vi "RestartSafety.vi"(0 "Universal Robot.lvclass in":refnum<class "Universal Robot.lvclass">, 5 "error in (no error)":errorcluster) -> (14 "Universal Robot.lvclass out":refnum<class "Universal Robot.lvclass">, 19 "error out":errorcluster)   [LabVIEW 2019, in "Universal Robot.lvclass"]
uses:
  Universal Robot.lvclass
  Universal Robot.lvclass/Universal Robot.ctl
  SafetyStatus.ctl
  Client Interfaces/Dashboard Server/Dashboard Server.lvclass
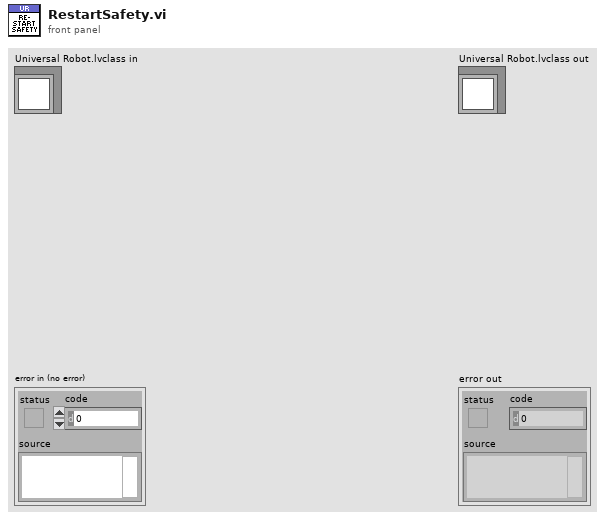
[diagram p1: front panel]
types:
  T1 = typedef "Universal Robot.lvclass/SafetyStatus.ctl" = enum16{"INVALID", "NORMAL", "REDUCED", "PROTECTIVE_STOP", "RECOVERY", "SAFEGUARD_STOP", "SYSTEM_EMERGENCY_STOP", "ROBOT_EMERGENCY_STOP", "VIOLATION", "FAULT", "AUTOMATIC_MODE_SAFEGAURD_STOP", "SYSTEM_THREE_POSITION_ENABLING_STOP"}
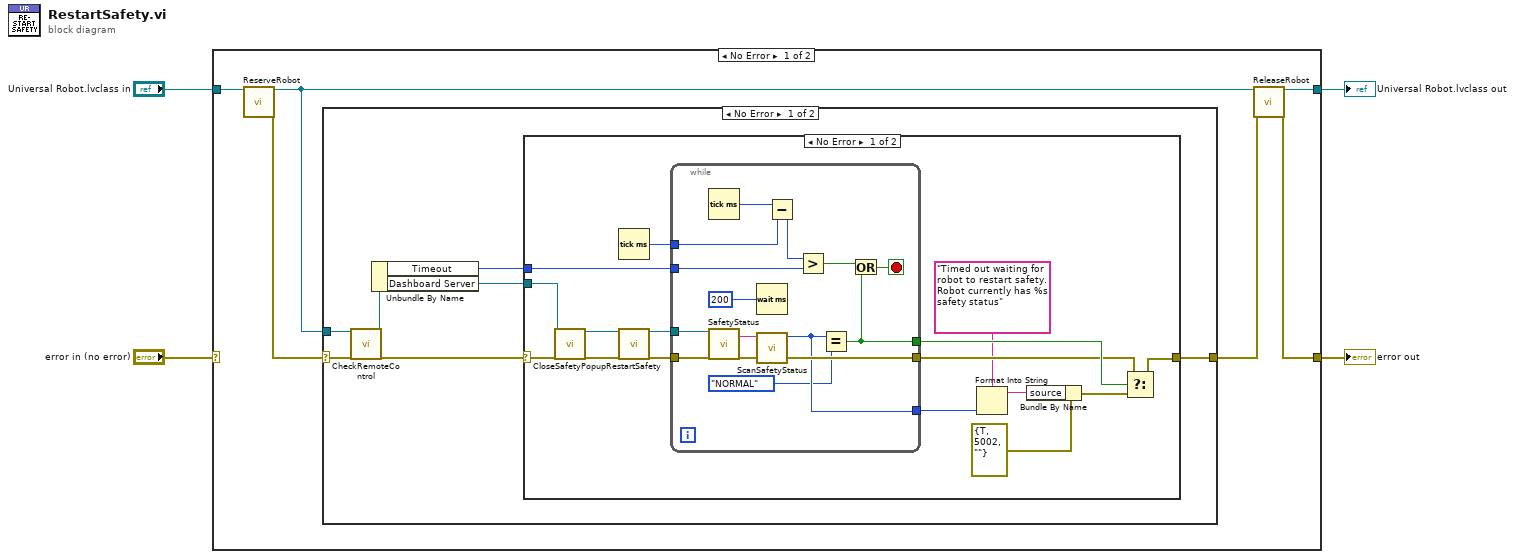
[diagram p0: block diagram]
diagram:
  n1 = case shown="No Error" "error in (no error)" {
    selector: "error in (no error)" -> [_ w51]
    tunnel: [w8 w51] -> w3
    tunnel: "Universal Robot.lvclass in" -> [w7 w50]
    tunnel: [w10 w50] -> w1
    frame No Error {
      n2 = call "ReserveRobot.vi"("Universal Robot.lvclass in"=w7) -> ("Universal Robot.lvclass out"=w6:refnum<class "Universal Robot.lvclass">, "error out"=w5:errorcluster)  [unwired: 17 in]
      n3 = case shown="No Error" w5 {
        selector: w5 -> [w11 w49]
        tunnel: [w13 w49] -> w9
        tunnel: w6 -> [w12 _]
        frame No Error {
          n4 = call-dynamic "CheckRemoteControl.vi"("Universal Robot.lvclass in"=w12, "error in (no error)"=w11) -> ("Universal Robot.lvclass out"=w17:refnum<class "Universal Robot.lvclass">, "error out"=w14:errorcluster)  [unwired: 16 in]
          n5 = Unbundle By Name(w17) -> ("Timeout"=w15:u32, "Dashboard Server"=w16:refnum<class "Dashboard Server.lvclass">)
          n6 = case shown="No Error" w14 {
            selector: w14 -> [w23 w48]
            tunnel: [w33 w48] -> w13
            tunnel: w16 -> [w22 _]
            tunnel: w15 -> [w32 _]
            frame No Error {
              n7 = call-dynamic "CloseSafetyPopup.vi"("DashboardServer in"=w22, "error in (no error)"=w23) -> ("DashboardServer out"=w21:refnum<class "Dashboard Server.lvclass">, "error out"=w20:errorcluster)  [unwired: 15 in, 1 out]
              n8 = Tick Count (ms)() -> (millisecond timer value=w31:u32)
              n9 = call-dynamic "RestartSafety.vi"("DashboardServer in"=w21, "error in (no error)"=w20) -> ("DashboardServer out"=w19:refnum<class "Dashboard Server.lvclass">, "error out"=w18:errorcluster)  [unwired: 15 in, 1 out]
              n10 = while {
                tunnel: [w39] -> w29
                tunnel: w32 -> [w46]
                tunnel: w31 -> [w45]
                tunnel: [w40] -> w30
                tunnel: [w35] -> w28
                tunnel: w19 -> [w38]
                tunnel: w18 -> [w37]
                stop <- w41 stop-if-true
                n11 = Tick Count (ms)() -> (millisecond timer value=w44:u32)
                n12 = call-dynamic "SafetyStatus.vi"("DashboardServer in"=w38, "error in (no error)"=w37) -> ("safetyStatus"=w36:string, "error out"=w39:errorcluster)  [unwired: 15 in, 1 out]
                n13 = Wait (ms)(milliseconds to wait=u32 200) -> ()  [unwired: 1 out]
                n14 = call "ScanSafetyStatus.vi"("safetyStatus in"=w36) -> ("safetyStatus out"=w35:T1)  [unwired: 10 in]
                n15 = Subtract(x=w44, y=w45) -> (x-y=w43:u32)
                n16 = Greater?(x=w43, y=w46) -> (0:w42:bool)
                n17 = Equal?(x=w35, y=SafetyStatus."NORMAL") -> (x = y?=w40:bool)
                n18 = Or(x=w42, y=w40) -> (x .or. y?=w41:bool)
              }
              n19 = Format Into String(format string="Timed out waiting for robot to restart safety. Robot currently has %s safety status", w28) -> (resulting string=w26:string)  [unwired: 2 in, 1 out]
              n20 = Bundle By Name(cluster=errorcluster {"status"=TRUE, "code"=5002, "source"=""} ("error constant"), "source"=w26) -> (w25:errorcluster)
              n21 = Select(t=w29, s=w30, f=w25) -> (s? t:f=w33:errorcluster)
            }
            frame Error {
            }
          }
        }
        frame Error {
        }
      }
      n22 = call "ReleaseRobot.vi"("Universal Robot.lvclass in"=w6, "error in (no error)"=w9) -> ("Universal Robot.lvclass out"=w10:refnum<class "Universal Robot.lvclass">, "error out"=w8:errorcluster)  [unwired: 16 in]
    }
    frame Error {
    }
  }
  "error out" <- w3
  "Universal Robot.lvclass out" <- w1
